vi "INIT_path.vi"(8 "error in (no error)":errorcluster caption="错误输入（无错误）", 11 "Path_management 输入":refnum<class "Path_management.lvclass">) -> (0 "error out":errorcluster caption="错误输出", 3 "Path_management 输出":refnum<class "Path_management.lvclass">)   [LabVIEW 2025, in "Path_management.lvclass"]
uses:
  Path_management.lvclass
panel:
  # "欢迎━(*｀?′*)ノ亻!\n使用这个超级好用的路径管理类"
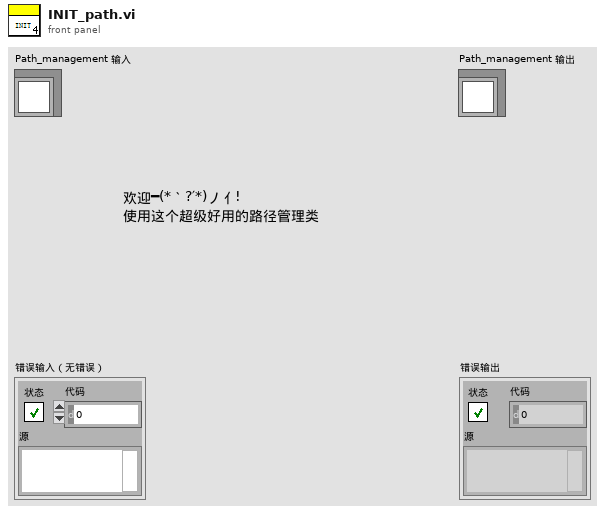
[diagram p1: front panel]
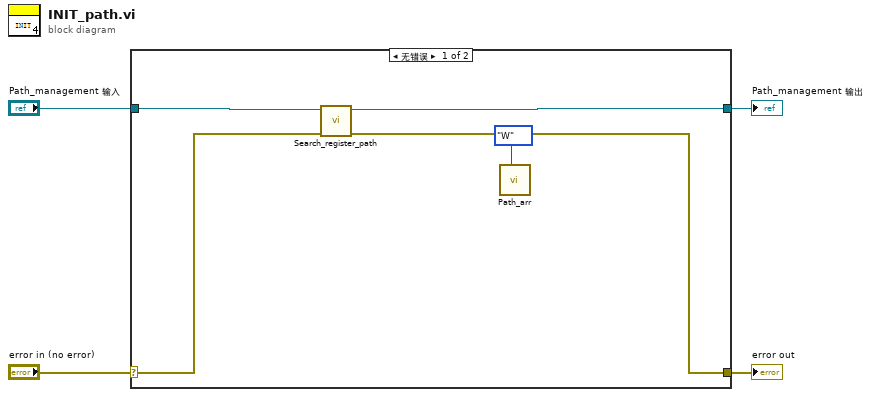
[diagram p0: block diagram]
diagram:
  n1 = case shown="无错误" "error in (no error)" {
    selector: "error in (no error)" -> [w7 w11]
    tunnel: [w6 w11] -> w3
    tunnel: [w5 w10] -> w1
    tunnel: "Path_management 输入" -> [w8 w10]
    frame No Error {
      n2 = call-dynamic "Search_register_path.vi"("error in (no error)"=w7, "Path_management 输入"=w8) -> ("error out"=w6:errorcluster, "Path_management 输出"=w5:refnum<class "Path_management.lvclass">)  [unwired: 7 in, 1 out]
      n3 = call "Path_arr.vi"("MJ"=enum16{"R", "W"}."W") -> ()  [unwired: 10 in, 1 out]
    }
    frame Error {
    }
  }
  "error out" <- w3
  "Path_management 输出" <- w1
